vi "Load_Timing_Config.vi"(11 "INI File Path":path=path "C:/YOUXI/dazuoye/Config/P1_Runtime.ini" caption="配置文件的路径") -> (1 "INI Load Error":errorcluster caption="错误输出", 2 "Loaded Countdown (s)":dbl=30.0 caption="值", 3 "Loaded Suspect (s)":dbl=5.0 caption="值")   [LabVIEW 2020]
uses:
  <vilib>/Utility/config.llb/Open Config Data.vi
  <vilib>/Utility/config.llb/Read Key (Double).vi
  <vilib>/Utility/config.llb/Close Config Data.vi
  <vilib>/Utility/config.llb/NI_LVConfig.lvlib
panel:
  out "Countdown Key Found":bool caption="已找到？"
  out "Suspect Key Found":bool caption="已找到？"
  in  "Default Countdown (s)":dbl=30.0 caption="默认值"
  in  "Default Suspect (s)":dbl=5.0 caption="默认值"
  in  "Countdown Key":string="CountdownSeconds" caption="键"
  in  "Suspect Key":string="SuspectDelaySeconds" caption="键"
  in  "INI Section":string="Timing" caption="段"
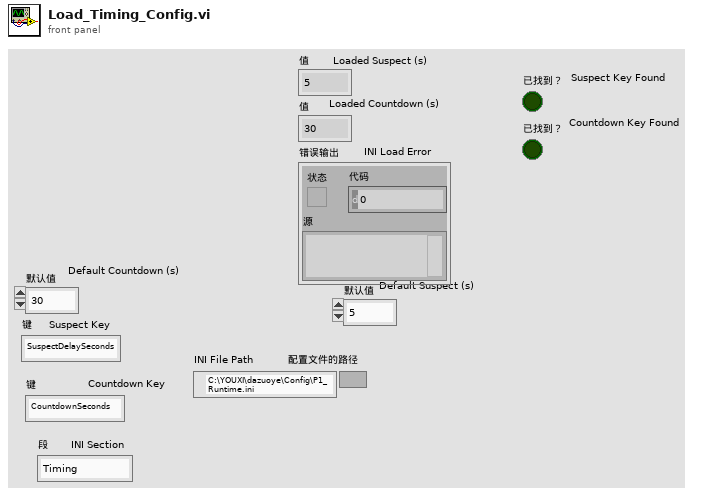
[diagram p1: front panel]
types:
  T1 = typedef "NI_LVConfig.lvlib/Config Data RefNum.ctl" = refnum<k1>
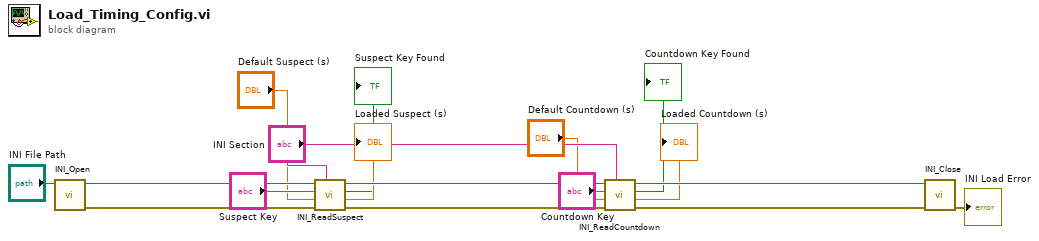
[diagram p0: block diagram]
diagram:
  n1 = call "INI_Open"("configuration file path"="INI File Path") -> ("error out"=w16:errorcluster, "refnum"=w17:T1)  [unwired: 8 in, 1 out]
  n2 = call "INI_ReadSuspect"("section"="INI Section", "error in (no error)"=w16, "default value"="Default Suspect (s)", "key"="Suspect Key", "refnum"=w17) -> ("error out"=w14:errorcluster, "value"=→"Loaded Suspect (s)":dbl, "found?"=→"Suspect Key Found":bool, "refnum out"=w15:T1)  [unwired: 3 in]
  n3 = call "INI_ReadCountdown"("section"="INI Section", "error in (no error)"=w14, "default value"="Default Countdown (s)", "key"="Countdown Key", "refnum"=w15) -> ("error out"=w12:errorcluster, "value"=→"Loaded Countdown (s)":dbl, "found?"=→"Countdown Key Found":bool, "refnum out"=w13:T1)  [unwired: 3 in]
  n4 = call "INI_Close"("error in (no error)"=w12, "refnum"=w13) -> ("error out"=→"INI Load Error":errorcluster)  [unwired: 8 in, 1 out]
